vi "VIH HelpGen - Build Named Numeric Ctrl Value Table - Find Dscr Index.vi"(6 "Class":enum16{"Enum", "Ring"}(ring), 8 "Strings":string[](array[string]), 9 "Values":ext[](array[numeric]), 10 "String":string, 11 "Value":ext) -> (0 "Index":i32)   [LabVIEW 2014]
doc: "::: VI Helpeks :::\nCopyright (c) 2000-2026 Konstantin Shifershteyn. All rights reserved."
panel:
  # "VI Helpeks\nCopyright (c) 2012-2026 Konstantin Shifershteyn"
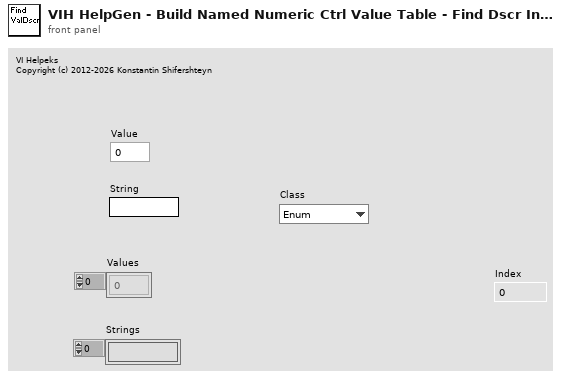
[diagram p1: front panel]
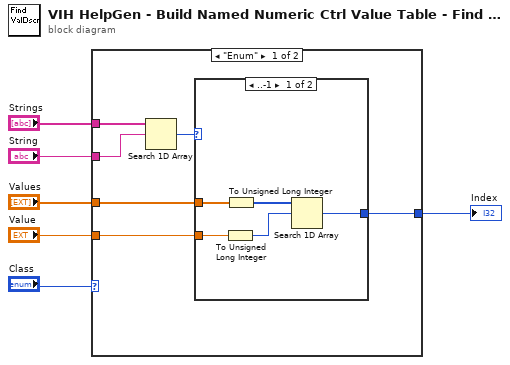
[diagram p0: block diagram]
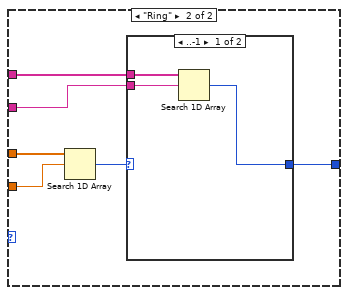
[diagram p3: hidden frame]
diagram:
  n1 = case shown="\"Enum\"" "Class" {
    tunnel: "Strings" -> [w12 w20]
    tunnel: "String" -> [w11 w19]
    tunnel: "Values" -> [w9 w24]
    tunnel: "Value" -> [w8 w23]
    tunnel: [w7 w21] -> w2
    frame "Enum" {
      n2 = Search 1D Array(1D array=w12, element=w11) -> (index of element=w10:i32)  [unwired: 1 in]
      n3 = case shown="..-1" w10 {
        selector: w10 -> [_ w18]
        tunnel: w9 -> [w17 _]
        tunnel: w8 -> [w16 _]
        tunnel: [w15 w18] -> w7
        frame ..-1 {
          n4 = To Unsigned Long Integer(number=w16) -> (unsigned 32bit integer=w13:u32)
          n5 = To Unsigned Long Integer(number=w17) -> (unsigned 32bit integer=w14:u32[])
          n6 = Search 1D Array(1D array=w14, element=w13) -> (index of element=w15:i32)  [unwired: 1 in]
        }
        frame 0.. {
        }
      }
    }
    frame "Ring" {
      n7 = Search 1D Array(1D array=w24, element=w23) -> (index of element=w22:i32)  [unwired: 1 in]
      n8 = case shown="..-1" w22 {
        selector: w22 -> [_ w28]
        tunnel: [w26 w28] -> w21
        tunnel: w20 -> [w27 _]
        tunnel: w19 -> [w25 _]
        frame ..-1 {
          n9 = Search 1D Array(1D array=w27, element=w25) -> (index of element=w26:i32)  [unwired: 1 in]
        }
        frame 0.. {
        }
      }
    }
  }
  "Index" <- w2
